vi "Distance measurement software - Main VI.vi"() -> ()   [LabVIEW 2025]
uses:
  Interpolation_Method.ctl
  state_enum.ctl
  <vilib>/gmath/NI_Gmath.lvlib
  <vilib>/Analysis/NI_AALBase.lvlib
panel:
  out "Alarm":bool
  out "Voltage":dbl
  out "Distance":dbl
  in  "File type":enum16{".csv", ".txt"}(ring)
  in  "Header string":string[][](array[string])
  in  "Save measurement file":bool
  out "Time [s] | Voltage [V] | Distance [cm]":dbl[][](array[numeric])
  out "Waveform Chart":cluster{"Numeric":dbl, dbl}(graph)
  out "Distance [cm] | Voltage [V]":dbl[][](array[numeric])
  in  "Interpolation Method used":T1
  in  "Stop Button":bool
  in  "Stop measurement":bool
  in  "Start measurement":bool
  in  "Calibrate":bool
  # "ALARM\n(under 40 cm)"
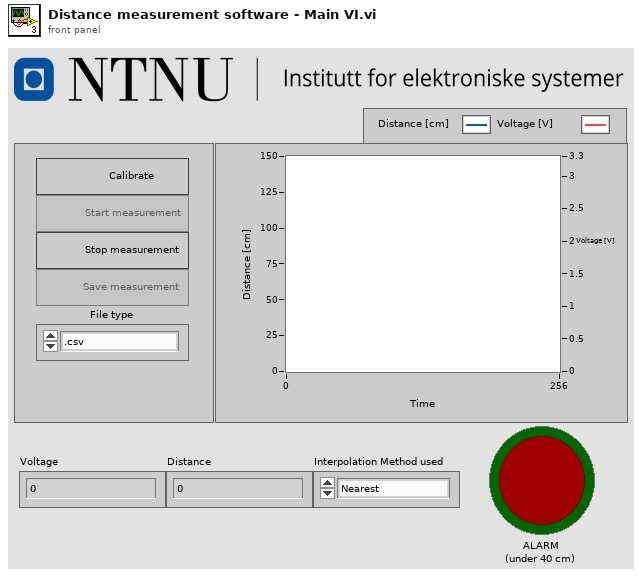
[diagram p1: front panel]
types:
  T1 = typedef "Interpolation_Method.ctl" = enum16{"Nearest", "Linear", "Spline", "Cubic Hermite", "Lagrange"}
  T2 = enum8{"Enabled", "Disabled", "Disabled and Grayed Out"}
  T3 = typedef "state_enum.ctl" = enum16{"Wait for event", "Calibrate", "Measure", "Save to file"}
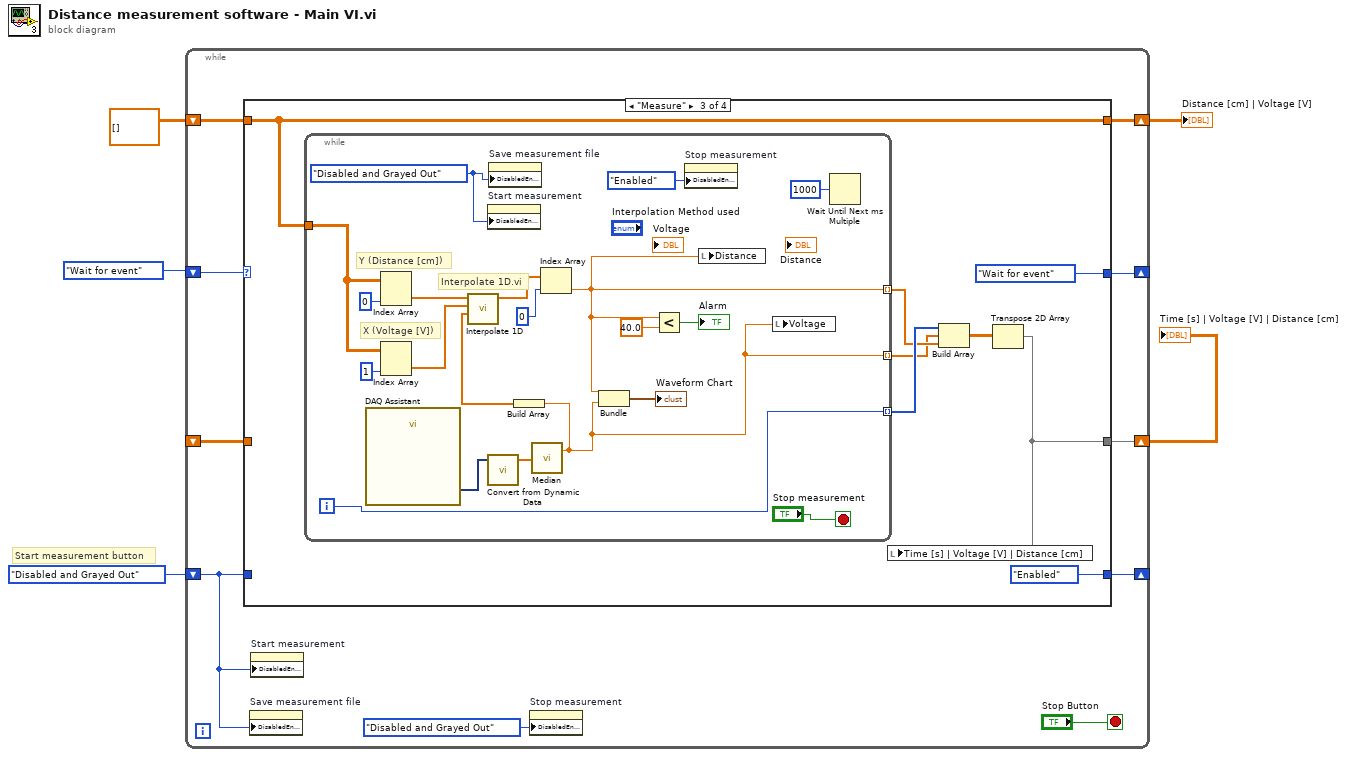
[diagram p0: block diagram]
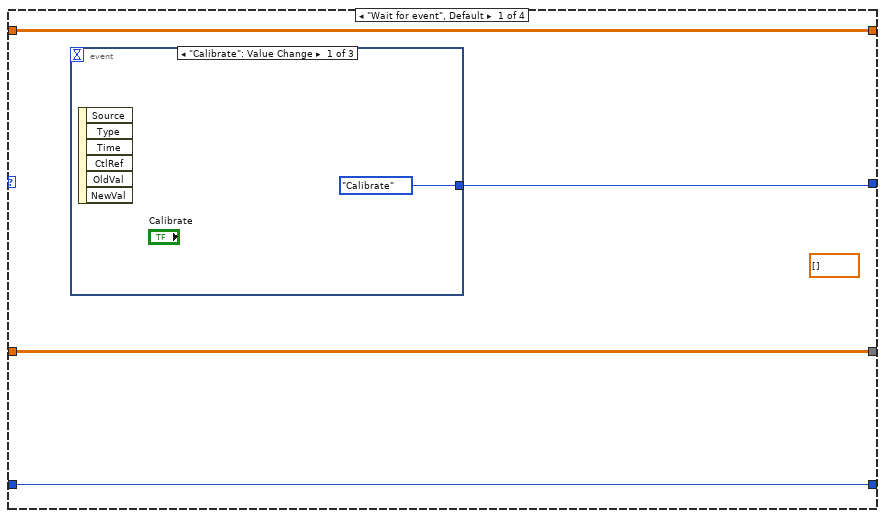
[diagram p2: hidden frame]
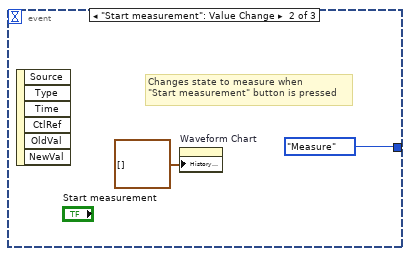
[diagram p3: hidden frame]
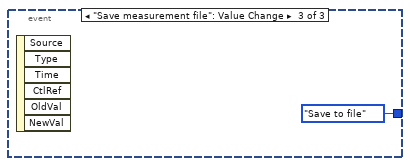
[diagram p4: hidden frame]
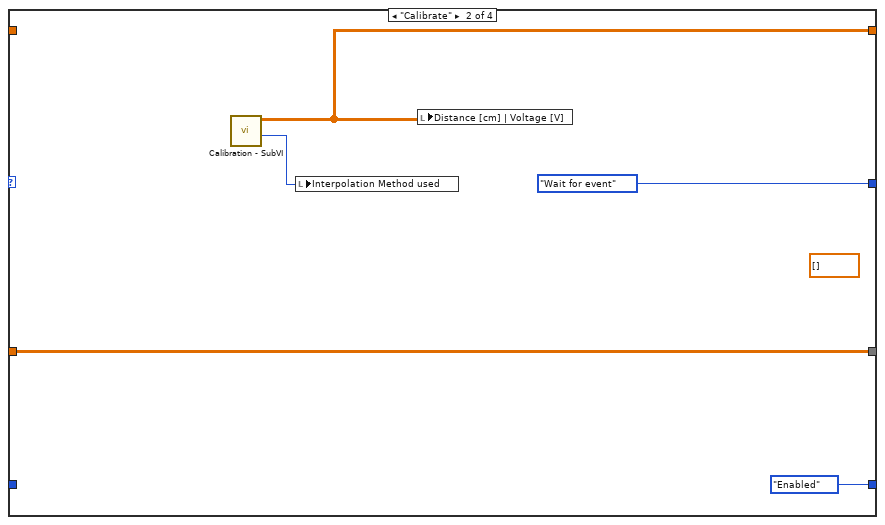
[diagram p5: hidden frame]
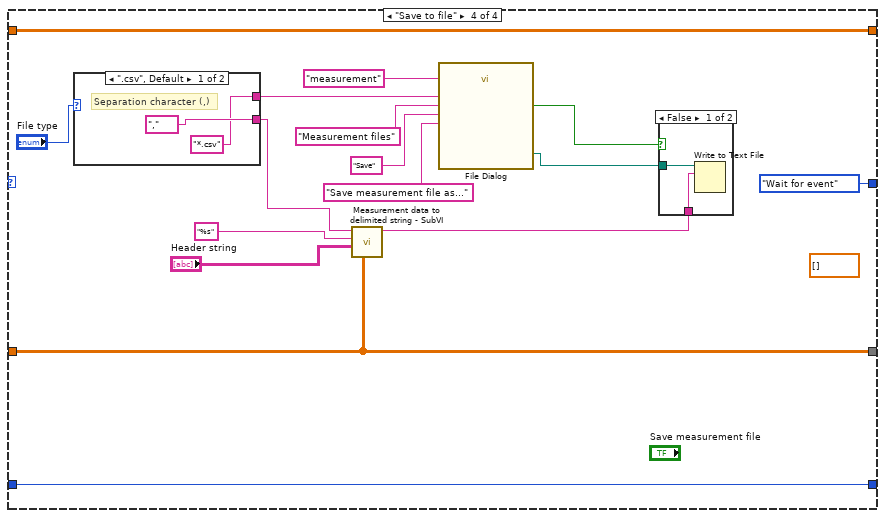
[diagram p6: hidden frame]
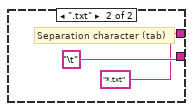
[diagram p8: hidden frame]
diagram:
  # "Start measurement button"
  n1 = while {
    shift-right: [w15] -> _
    shift-left: state_enum."Wait for event" -> [w14]
    shift-right: [w12] -> w4
    shift-left: dbl[][] [] ("Distance [cm] | Voltage [V]") -> [w11]
    shift-right: [w10] -> w2
    shift-left: _ -> [w9]
    shift-right: [w8] -> _
    shift-left: T2."Disabled and Grayed Out" ("Disabled") -> [w6]
    stop <- "Stop Button" stop-if-true
    n2 = case shown="\"Measure\"" w14 {
      tunnel: [w19 state_enum."Wait for event" state_enum."Wait for event" state_enum."Wait for event"] -> w15
      tunnel: [w18 w26 w35 w64] -> w12
      tunnel: w11 -> [w18 _ w35 w64]
      tunnel: [w17 w25 w31 w63] -> w10
      tunnel: w9 -> [w17 w25 _ w63]
      tunnel: [w16 T2."Enabled" ("Disabled") T2."Enabled" ("Disabled") w57] -> w8
      tunnel: w6 -> [w16 _ _ w57]
      frame "Wait for event", Default {
        (unwired) dbl[] []
        n3 = event shown="[0] \"Calibrate\": Value Change" {
          selector: _ -> [_ _ _]
          dyn-events: _ -> [_ _ _]
          timeout: _ -> [_ _ _]
          tunnel: [state_enum."Calibrate" state_enum."Measure" state_enum."Save to file"] -> w19
          event "Calibrate": Value Change {
            n4 = event-data() -> ()  [unwired: 1 in, 6 out]
          }
          event "Start measurement": Value Change {
            # "Changes state to measure when \n\"Start measurement\" button is pressed"
            n5 = event-data() -> ()  [unwired: 1 in, 6 out]
            n6 = property on="Waveform Chart" class="WFChart (strict)"("History Data"=cluster{"Numeric":dbl, dbl}[] []) -> ()  [unwired: 2 in, 2 out]
          }
          event "Save measurement file": Value Change {
            n7 = event-data() -> ()  [unwired: 1 in, 6 out]
          }
        }
      }
      frame "Calibrate" {
        (unwired) dbl[] []
        n8 = call "Calibration - SubVI.vi"() -> ("Interpolation Method"=w28:T1, "Distance [cm] | Voltage [V]"=w26:dbl[][])  [unwired: 10 in]
        n9 = local write "Interpolation Method used"(w28) -> ()
        n10 = local write "Distance [cm] | Voltage [V]"(w26) -> ()
      }
      frame "Measure" {
        n11 = while {
          tunnel: w35 -> [w51]
          tunnel: [w39] -> w32 mode=indexing
          tunnel: [w41] -> w33 mode=indexing
          tunnel: [w40] -> w29 mode=indexing
          i -> [w41]
          stop <- "Stop measurement" stop-if-true
          w47 = T2."Disabled and Grayed Out" ("Disabled")
          # "Interpolate 1D.vi"
          # "X (Voltage [V])"
          # "Y (Distance [cm])"
          n12 = call "DAQ Assistant"() -> ("data"=w46:dynamicdata)  [unwired: 17 in, 2 out]
          n13 = Index Array(array=w51, index (col)=0 ("disabled index (col)")) -> (element=w52:dbl[])  [unwired: 1 in]
          n14 = Index Array(array=w51, index (col)=1 ("disabled index (col)")) -> (element=w53:dbl[])  [unwired: 1 in]
          n15 = property on="Start measurement" class="Bool"("DisabledEnum"=w47) -> ()  [unwired: 2 in, 2 out]
          n16 = call "Convert from Dynamic Data"("Dynamic Data Type"=w46) -> ("Array"=w44:dbl[])  [unwired: 3 in]
          n17 = property on="Save measurement file" class="Bool"("DisabledEnum"=w47) -> ()  [unwired: 2 in, 2 out]
          n18 = call <vilib>:"Median.vi"("X"=w44) -> ("median"=w40:dbl)  [unwired: 1 out]
          n19 = Build Array(w40) -> (w43:dbl[])
          n20 = call <vilib>:"Interpolate 1D.vi"("xi"=w43, "X"=w53, "Y"=w52) -> ("yi"=w50:dbl[])  [unwired: 6 in, 2 out]
          n21 = Index Array(array=w50, index=0) -> (element=w39:dbl)
          n22 = Bundle("Numeric"=w39, "median"=w40) -> (→"Waveform Chart":cluster{"Numeric":dbl, "median":dbl})  [unwired: 1 in]
          n23 = Less?(x=w39, y=40.0) -> (x < y?=→"Alarm":bool)
          n24 = property on="Stop measurement" class="Bool"("DisabledEnum"=T2."Enabled" ("Disabled")) -> ()  [unwired: 2 in, 2 out]
          n25 = local write "Distance"(w39) -> ()
          n26 = local write "Voltage"(w40) -> ()
          n27 = Wait Until Next ms Multiple(millisecond multiple=u32 1000) -> ()  [unwired: 1 out]
        }
        n28 = Build Array(w33, w29, w32) -> (w34:dbl[][])
        n29 = Transpose 2D Array(2D array=w34) -> (transposed array=w31:dbl[][])
        n30 = local write "Time [s] | Voltage [V] | Distance [cm]"(w31) -> ()
      }
      frame "Save to file" {
        (unwired) dbl[] []
        n31 = case shown="\".csv\", Default" "File type" {
          tunnel: ["," "\t"] -> w61
          tunnel: ["*.csv" "*.txt"] -> w60
          frame ".csv", Default {
            # "Separation character (,)"
          }
          frame ".txt" {
            # "Separation character (tab)"
          }
        }
        n32 = call "Measurement data to delimited string - SubVI.vi"("Measurement data"=w63, "Header title string"="Header string", "Header format string"="%s" ("format string"), "Delimiter in"=w61) -> ("File string out"=w67:string)  [unwired: 7 in]
        n33 = call "File Dialog"("prompt"="Save measurement file as...", "button label"="Save", "default name"="measurement", "pattern (all files)"=w60, "pattern label"="Measurement files") -> ("selected path"=w59:path, "cancelled"=w58:bool)  [unwired: 7 in, 2 out]
        n34 = case shown="False" w58 {
          tunnel: w67 -> [w74 _]
          tunnel: w59 -> [w73 _]
          frame False {
            n35 = Write to Text File(file (use dialog)=w73, text=w74) -> ()  [unwired: 2 in, 3 out]
          }
          frame True {
          }
        }
      }
    }
    n36 = property on="Save measurement file" class="Bool"("DisabledEnum"=w6) -> ()  [unwired: 2 in, 2 out]
    n37 = property on="Start measurement" class="Bool"("DisabledEnum"=w6) -> ()  [unwired: 2 in, 2 out]
    n38 = property on="Stop measurement" class="Bool"("DisabledEnum"=T2."Disabled and Grayed Out" ("Disabled")) -> ()  [unwired: 2 in, 2 out]
  }
  "Distance [cm] | Voltage [V]" <- w4
  "Time [s] | Voltage [V] | Distance [cm]" <- w2
